vi "Write Device ID.vi"(8 "error in (no error)":errorcluster, 10 "Relay ID":T1 {"Serial Number" format="%06x"}, 11 "Device":string="hidraw0") -> (0 "error out":errorcluster)   [LabVIEW 2021, in "USB Relay Control.lvlib"]
uses:
  USB Relay Control.lvlib
  typedef/Relay ID.ctl
  typedef/Read Write.ctl
  typedef/Errors.ctl
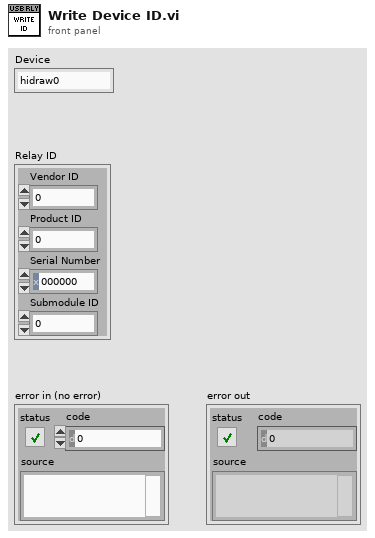
[diagram p1: front panel]
types:
  T1 = typedef "USB Relay Control.lvlib/Relay ID.ctl" = cluster{"Vendor ID":u8, "Product ID":u8, "Serial Number":u32, "Submodule ID":u8}
  T2 = typedef "USB Relay Control.lvlib/Errors.ctl" = enum16{"Invalid ID", "Failed to write ID"}
  T3 = typedef "USB Relay Control.lvlib/Read Write.ctl" = enum8{"Read", "Write"}
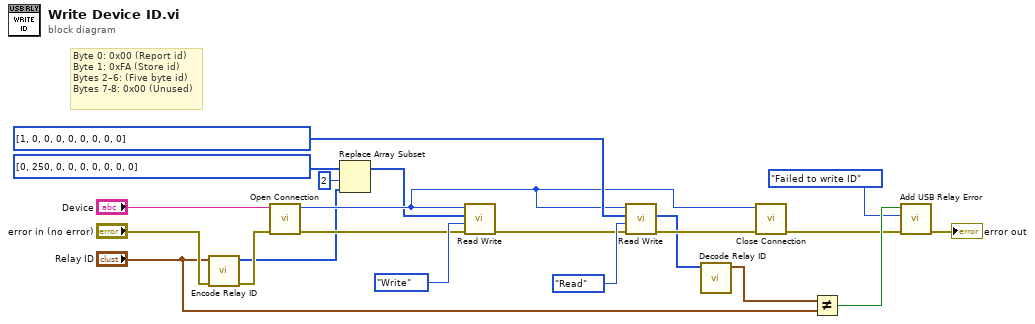
[diagram p0: block diagram]
diagram:
  # "Byte 0: 0x00 (Report id)\nByte 1: 0xFA (Store id)\nBytes 2–6: (Five byte id)\nBytes 7-8: 0x00 (Unused)"
  n1 = call "Encode Relay ID.vi"("error in (no error)"="error in (no error)", "Relay ID"="Relay ID") -> ("error out"=w12:errorcluster, "Encoded ID"=w8:u8[])  [unwired: 8 in]
  n2 = call "Open Connection.vi"("error in (no error)"=w12, "Device"="Device") -> ("error out"=w13:errorcluster, "HID RAW Reference"=w16:i32)  [unwired: 8 in]
  n3 = Replace Array Subset(array=u8[] [0, 250, 0, 0, 0, 0, 0, 0, 0] ("Buffer In"), new element=w8, index=2) -> (w7:u8[])
  n4 = call "Read Write.vi"("error in (no error)"=w13, "RW"=Read_Write."Write", "Buffer In"=w7, "HID RAW Reference"=w16) -> ("error out"=w17:errorcluster)  [unwired: 6 in, 1 out]
  n5 = call "Read Write.vi"("error in (no error)"=w17, "RW"=Read_Write."Read", "Buffer In"=u8[] [1, 0, 0, 0, 0, 0, 0, 0, 0], "HID RAW Reference"=w16) -> ("error out"=w21:errorcluster, "Buffer Out"=w14:u8[])  [unwired: 6 in]
  n6 = call "Decode Relay ID.vi"("Encoded ID"=w14) -> ("Relay ID"=w6:T1)  [unwired: 10 in]
  n7 = call "Close Connection.vi"("error in (no error)"=w21, "HID RAW Reference"=w16) -> ("error out"=w3:errorcluster)  [unwired: 9 in]
  n8 = Not Equal?(x=w6, y="Relay ID") -> (x != y?=w4:bool)
  n9 = call "Add USB Relay Error.vi"("error in (no error)"=w3, "Error"=Errors."Failed to write ID", "Insert Error"=w4) -> ("error out"=→"error out":errorcluster)  [unwired: 8 in]
